vi "Camera Messenger.vi"(0 "Notifier Name":string, 1 "Binning":u16, 2 "General Camera Actions":T3, 5 "Exposure Time (s)":dbl, 7 "Save Path":path, 9 "No. of Frames":u32, 11 "Camera ROI":T1, 12 "Cooler On/Off":bool, 13 "Defect Correction On/Off":bool, 14 "Fan On/Off":bool) -> (3 "Current Exposure Time (s)":dbl, 4 "Notifier Name Dup":string, 6 "Running?":bool, 8 "Camera ROI":T1, 10 "Current Frame":u32, 15 "Image Ref":T2)   [LabVIEW 2021]
uses:
  Camera Controls/Generic Camera Actions.ctl
  Camera Controls/Generic Camera ROI.ctl
  <vilib>/vision/Image Controls.llb/IMAQ Image.ctl
  Hardware Configuration/Hardware Configuration Controls/Company.ctl
  Hamamatsu/Orca Flash/Orca Flash Controls/Orca Flash ROI.ctl
  Hamamatsu/Orca Flash/Orca Flash Controls/Orca Flash Parameters.ctl
  Hamamatsu/Orca Flash/Orca Flash Controls/Orca Flash Parameter List.ctl
  Hamamatsu/Orca Flash/Orca Flash Controls/Orca Flash Actions.ctl
  IDS/IDS Controls/IDS ROI.ctl
  IDS/IDS Controls/IDS Parameters.ctl
  IDS/IDS Controls/IDS Parameter List.ctl
  IDS/IDS Controls/IDS Actions.ctl
  Ximea/Ximea Controls/Ximea ROI.ctl
  Ximea/Ximea Controls/Ximea Parameters.ctl
  Ximea/Ximea Controls/Ximea Parameter List.ctl
  Ximea/Ximea Controls/Ximea Actions.ctl
  Photometrics/Prime BSI/R Cubed SITK/Prime BSI R3 Controls/Prime R3 ROI.ctl
  Photometrics/Prime BSI/R Cubed SITK/Prime BSI R3 Controls/Prime R3 Parameters.ctl
  Photometrics/Prime BSI/R Cubed SITK/Prime BSI R3 Controls/Prime R3 Parameter List.ctl
  Photometrics/Prime BSI/R Cubed SITK/Prime BSI R3 Controls/Prime R3 Actions.ctl
  Camera Controls/Camera IMAQ Key Info.ctl
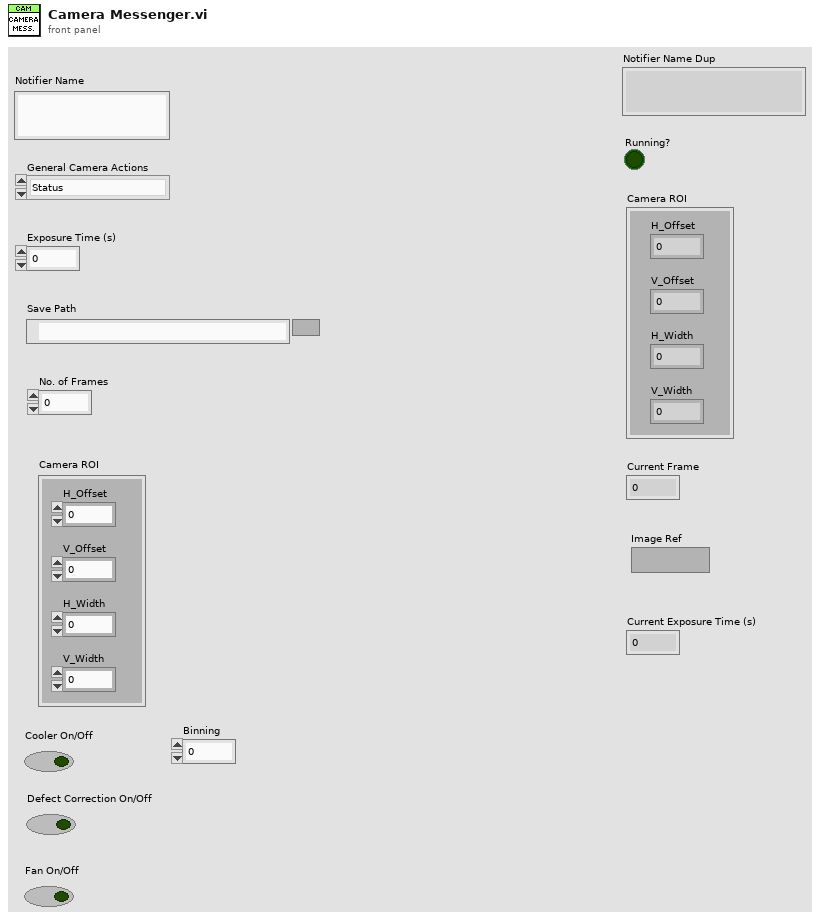
[diagram p1: front panel]
types:
  T1 = typedef "Generic Camera ROI.ctl" = cluster{"H_Offset":u16, "V_Offset":u16, "H_Width":u16, "V_Width":u16}
  T2 = typedef "IMAQ Image.ctl" = refnum<image>
  T3 = typedef "Generic Camera Actions.ctl" = enum16{"Status", "Live Preview", "Capture", "Abort", "Set Exposure Time (s)", "Get Exposure Time (s)", "Set Gain", "Get Gain", "Set Gamma", "Get Gamma", "Record Settings", "Set ROI", "Get ROI", "Binning", "Defect Correction On/Off", "Cooler On/Off", "Fan On/Off", "Quit"}
  T4 = typedef "Company.ctl" = enum16{"AA Opto Electronic", "ASI", "Coherent", "CVI", "DAQmx", "Hamamatsu", "IDS", "Ximea", "Mad City Labs", "Marzhauser", "Measurement Computing", "MPB Com", "Photometrics", "PI", "Prior", "Thorlabs"}
  T5 = typedef "Orca Flash Parameters.ctl" = cluster{"Value":dbl, "Orca Flash Parameters":T6}
  T6 = typedef "Orca Flash Parameter List.ctl" = u32
  T7 = typedef "Orca Flash ROI.ctl" = cluster{"H Offset":i32, "V Offset":i32, "H Width":i32, "V Width":i32}
  T8 = typedef "Orca Flash Actions.ctl" = enum16{"IDLE", "PREVIEW", "RECORD", "Send Trigger", "SOFT TRIGGER", "Record Settings", "SETPARAM", "GETPARAM", "SETROI", "GETROI", "PROGRESSIVE MODE", "AREA MODE", "STATUS", "QUIT"}
  T9 = typedef "IDS Parameter List.ctl" = enum16{"Exposure Time (s)", "Binning", "Gain", "Gamma"}
  T10 = typedef "IDS Parameters.ctl" = cluster{"Parameter":T9, "Value":dbl}
  T11 = typedef "IDS ROI.ctl" = cluster{"H Offset":i32, "V Offset":i32, "H Width":i32, "V Width":i32}
  T12 = typedef "IDS Actions.ctl" = enum16{"Error Check", "Initialize", "Preview", "Record", "Abort", "Record Settings", "Set Parameter", "Get Parameter", "Set ROI", "Get ROI", "Status", "Quit"}
  T13 = typedef "Ximea Parameter List.ctl" = enum16{"Exposure Time (s)", "Gain"}
  T14 = typedef "Ximea Parameters.ctl" = cluster{"Parameter":T13, "Value":sgl}
  T15 = typedef "Ximea ROI.ctl" = cluster{"H Offset":i32, "V Offset":i32, "H Width":i32, "V Width":i32}
  T16 = typedef "Ximea Actions.ctl" = enum16{"Idle", "Error Check", "Preview", "Record", "Soft Trigger", "Abort", "Record Settings", "Set Parameter", "Get Parameter", "Set ROI", "Get ROI", "Status", "Quit"}
  T17 = typedef "Prime R3 Parameter List.ctl" = enum16{"Exposure Time (s)"}
  T18 = typedef "Prime R3 Parameters.ctl" = cluster{"Parameter":T17, "Value":dbl}
  T19 = typedef "Prime R3 ROI.ctl" = cluster{"X Start":u32, "X End":u32, "X Bin":u32, "Y Start":u32, "Y End":u32, "Y Bin":u32}
  T20 = typedef "Prime R3 Actions.ctl" = enum16{"Error Check", "Initialize", "Preview", "Record", "Abort", "Record Settings", "Set Parameter", "Get Parameter", "Set ROI", "Get ROI", "Status", "Set Trigger", "Quit"}
  T21 = typedef "Camera IMAQ Key Info.ctl" = cluster{"Frame":u32, "Sensor Height":i32, "Sensor Width":i32, "ROI Height":i32, "ROI Width":i32, "ROI Enable?":bool, "Bit per Pixel":u8}
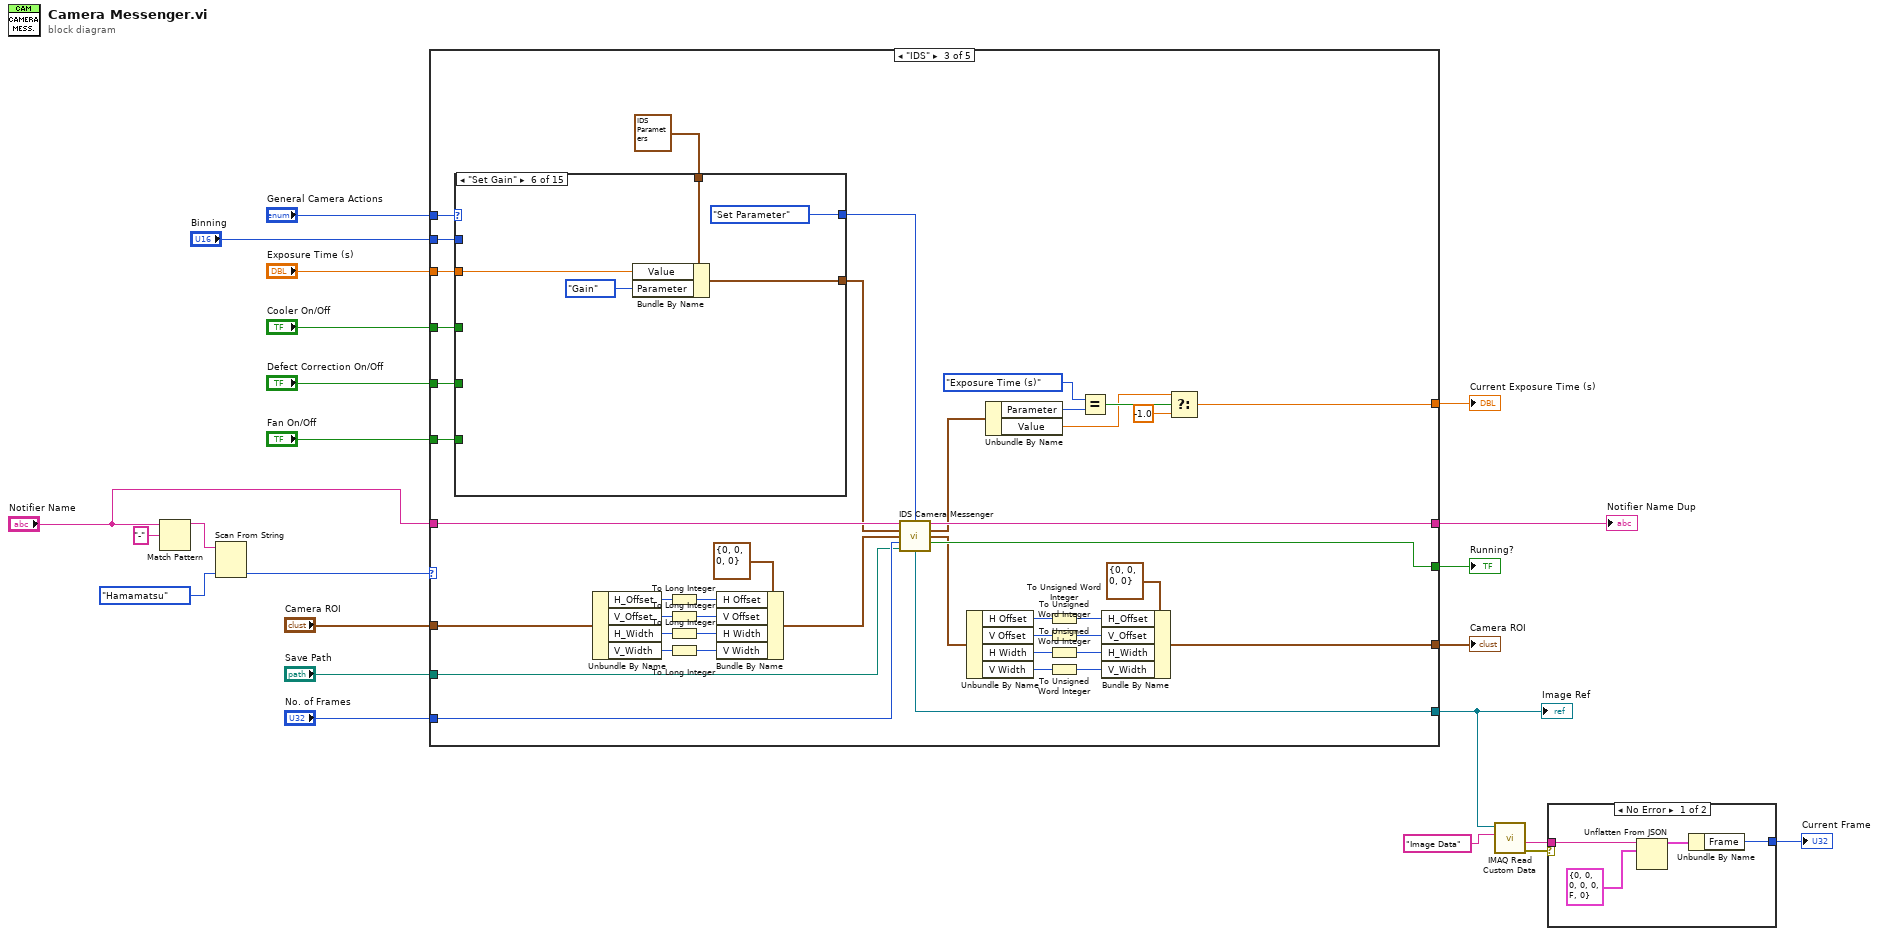
[diagram p0: block diagram]
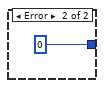
[diagram p2: hidden frame]
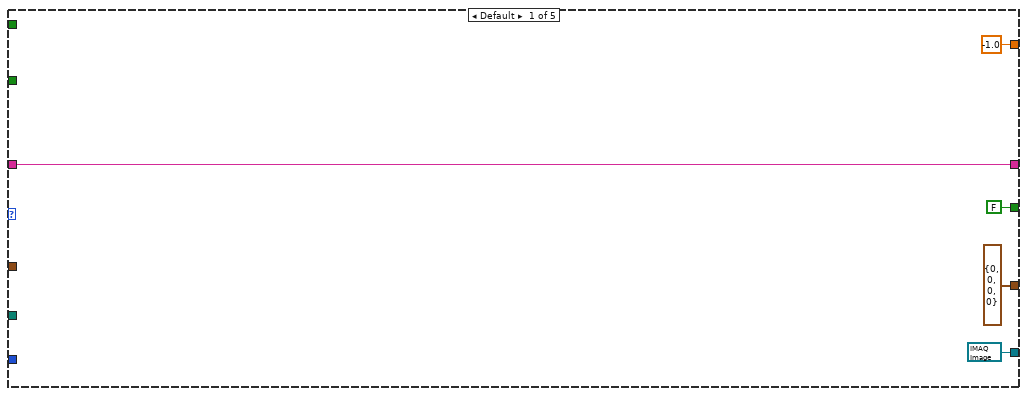
[diagram p3: hidden frame]
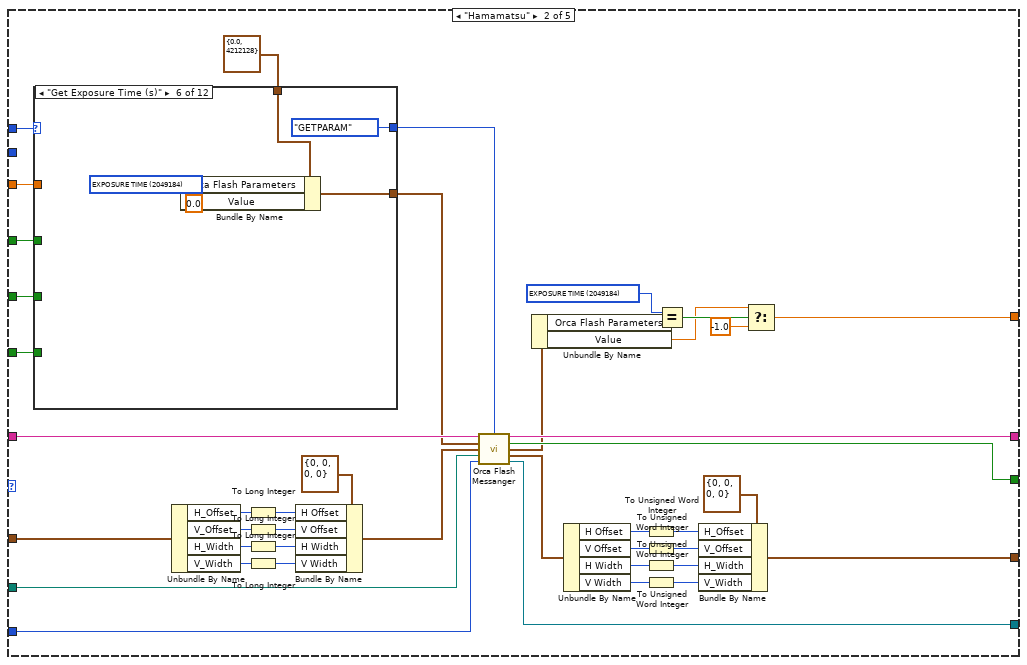
[diagram p4: hidden frame]
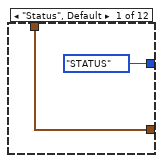
[diagram p5: hidden frame]
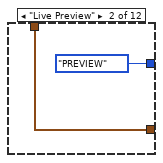
[diagram p6: hidden frame]
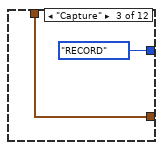
[diagram p7: hidden frame]
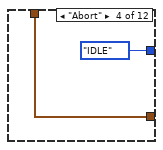
[diagram p8: hidden frame]
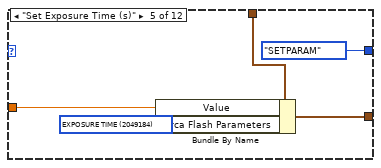
[diagram p9: hidden frame]
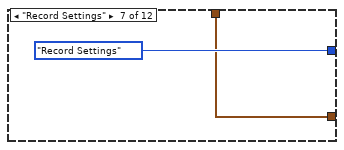
[diagram p10: hidden frame]
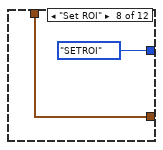
[diagram p11: hidden frame]
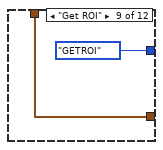
[diagram p12: hidden frame]
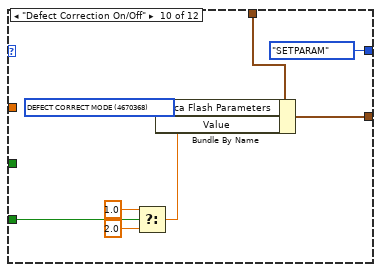
[diagram p13: hidden frame]
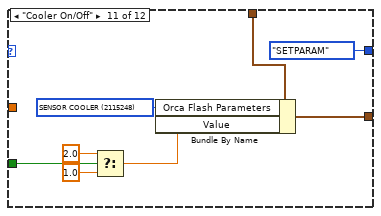
[diagram p14: hidden frame]
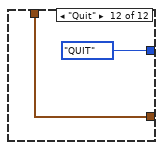
[diagram p15: hidden frame]
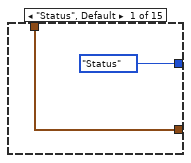
[diagram p16: hidden frame]
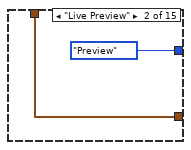
[diagram p17: hidden frame]
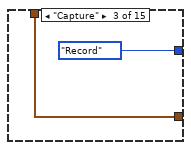
[diagram p18: hidden frame]
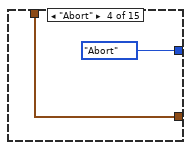
[diagram p19: hidden frame]
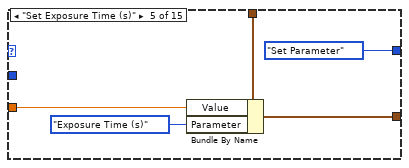
[diagram p20: hidden frame]
diagram:
  n1 = Match Pattern(string="Notifier Name", regular expression="-") -> (before substring=w20:string)  [unwired: 1 in, 3 out]
  n2 = Scan From String(input string=w20, default 1=Company."Hamamatsu" ("Company")) -> (output 1=w21:T4)  [unwired: 3 in, 3 out]
  n3 = case shown="\"IDS\"" w21 {
    tunnel: "Notifier Name" -> [w28 w71 w157 w246 w318]
    tunnel: "General Camera Actions" -> [_ w56 w142 w231 w311]
    tunnel: "No. of Frames" -> [_ w70 w156 w245 w317]
    tunnel: "Save Path" -> [_ w69 w155 w244 w289]
    tunnel: "Camera ROI" -> [_ w67 w153 w242 w315]
    tunnel: [w28 w57 w143 w232 w312] -> w15
    tunnel: "Exposure Time (s)" -> [_ w51 w138 w227 w307]
    tunnel: "Cooler On/Off" -> [_ w55 w141 w230 w310]
    tunnel: "Defect Correction On/Off" -> [_ w54 w140 w229 w309]
    tunnel: "Fan On/Off" -> [_ w53 w139 w228 w308]
    tunnel: [T2 refnum ("Image Ref") w48 w135 w224 w304] -> w6
    tunnel: [FALSE ("Running?") w47 w134 w223 w303] -> w10
    tunnel: [T1 {"H_Offset"=0, "V_Offset"=0, "H_Width"=0, "V_Width"=0} ("General Camera ROI") w36 w123 w212 w292] -> w9
    tunnel: [-1.0 ("f") w30 w115 w206 w274] -> w2
    tunnel: "Binning" -> [_ _ w114 _ _]
    frame Default {
    }
    frame "Hamamatsu" {
      w29 = T6 2049184 items=["SENSOR MODE"=4212128, "READOUT SPEED"=4211872, "READOUT DIRECTION"=4211904, "TRIGGER GLOBAL EXPOSURE"=2049680, "TRIGGER DELAY"=1066480, "SYNC READOUT SYSTEM BLANK"=1066528, "SENSOR COOLER"=2115248, "SENSOR COOLER STATUS"=2115280, "EXPOSURE TIME"=2049184, "DEFECT CORRECT MODE"=4670368, "BINNING"=4215968, "INTERNAL LINE SPEED"=4226000, "INTERNAL LINE INTERVAL"=4226016, "IMAGE PIXEL TYPE"=4343296, "NUMBER OF OUTPUT TRIGGER CONNECTOR"=1852320, "OUTPUT TRIGGER SOURCE[0]"=1852576, "OUTPUT TRIGGER SOURCE[1]"=1852832, "OUTPUT TRIGGER SOURCE[2]"=1853088, "OUTPUT TRIGGER POLARITY[0]"=1852592, "OUTPUT TRIGGER POLARITY[1]"=1852848, "OUTPUT TRIGGER POLARITY[2]"=1853104, "OUTPUT TRIGGER ACTIVE[0]"=1852608, "OUTPUT TRIGGER ACTIVE[1]"=1852864, "OUTPUT TRIGGER ACTIVE[2]"=1853120, "OUTPUT TRIGGER DELAY[0]"=1852624, "OUTPUT TRIGGER DELAY[1]"=1852880, "OUTPUT TRIGGER DELAY[2]"=1853136, "OUTPUT TRIGGER PERIOD[0]"=1852640, "OUTPUT TRIGGER PERIOD[1]"=1852896, "OUTPUT TRIGGER PERIOD[2]"=1853152, "OUTPUT TRIGGER KIND[0]"=1852656, "OUTPUT TRIGGER KIND[1]"=1852912, "OUTPUT TRIGGER KIND[2]"=1853168, "OUTPUT TRIGGER PRE HSYNC COUNT"=1852704] ("x")
      n4 = case shown="\"Get Exposure Time (s)\"" w56 {
        tunnel: w55 -> [_ _ _ _ _ _ _ _ _ _ w108 _]
        tunnel: w54 -> [_ _ _ _ _ _ _ _ _ w99 _ _]
        tunnel: w53 -> [_ _ _ _ _ _ _ _ _ _ _ _]
        tunnel: [Orca_Flash_Actions."STATUS" ("Camera Actions") Orca_Flash_Actions."PREVIEW" ("Camera Actions") Orca_Flash_Actions."RECORD" ("Camera Actions") Orca_Flash_Actions."IDLE" ("Camera Actions") Orca_Flash_Actions."SETPARAM" ("Camera Actions") Orca_Flash_Actions."GETPARAM" ("Camera Actions") Orca_Flash_Actions."Record Settings" ("Camera Actions") Orca_Flash_Actions."SETROI" ("Camera Actions") Orca_Flash_Actions."GETROI" ("Camera Actions") Orca_Flash_Actions."SETPARAM" ("Camera Actions") Orca_Flash_Actions."SETPARAM" ("Camera Actions") Orca_Flash_Actions."QUIT" ("Camera Actions")] -> w52
        tunnel: w51 -> [_ _ _ _ w83 _ _ _ _ _ _ _]
        tunnel: [w72 w74 w76 w78 w82 w88 w90 w92 w94 w101 w104 w113] -> w50
        tunnel: T5 {"Value"=0.0, "Orca Flash Parameters"=4212128} ("sCMOS Parameter") -> [w72 w74 w76 w78 w81 w89 w90 w92 w94 w102 w110 w113]
        frame "Status", Default {
        }
        frame "Live Preview" {
        }
        frame "Capture" {
        }
        frame "Abort" {
        }
        frame "Set Exposure Time (s)" {
          w80 = T6 2049184 items=["SENSOR MODE"=4212128, "READOUT SPEED"=4211872, "READOUT DIRECTION"=4211904, "TRIGGER GLOBAL EXPOSURE"=2049680, "TRIGGER DELAY"=1066480, "SYNC READOUT SYSTEM BLANK"=1066528, "SENSOR COOLER"=2115248, "SENSOR COOLER STATUS"=2115280, "EXPOSURE TIME"=2049184, "DEFECT CORRECT MODE"=4670368, "BINNING"=4215968, "INTERNAL LINE SPEED"=4226000, "INTERNAL LINE INTERVAL"=4226016, "IMAGE PIXEL TYPE"=4343296, "NUMBER OF OUTPUT TRIGGER CONNECTOR"=1852320, "OUTPUT TRIGGER SOURCE[0]"=1852576, "OUTPUT TRIGGER SOURCE[1]"=1852832, "OUTPUT TRIGGER SOURCE[2]"=1853088, "OUTPUT TRIGGER POLARITY[0]"=1852592, "OUTPUT TRIGGER POLARITY[1]"=1852848, "OUTPUT TRIGGER POLARITY[2]"=1853104, "OUTPUT TRIGGER ACTIVE[0]"=1852608, "OUTPUT TRIGGER ACTIVE[1]"=1852864, "OUTPUT TRIGGER ACTIVE[2]"=1853120, "OUTPUT TRIGGER DELAY[0]"=1852624, "OUTPUT TRIGGER DELAY[1]"=1852880, "OUTPUT TRIGGER DELAY[2]"=1853136, "OUTPUT TRIGGER PERIOD[0]"=1852640, "OUTPUT TRIGGER PERIOD[1]"=1852896, "OUTPUT TRIGGER PERIOD[2]"=1853152, "OUTPUT TRIGGER KIND[0]"=1852656, "OUTPUT TRIGGER KIND[1]"=1852912, "OUTPUT TRIGGER KIND[2]"=1853168, "OUTPUT TRIGGER PRE HSYNC COUNT"=1852704] ("Parameter")
          n5 = Bundle By Name(cluster=w81, "Value"=w83, "Orca Flash Parameters"=w80) -> (w82:T5)
        }
        frame "Get Exposure Time (s)" {
          w86 = T6 2049184 items=["SENSOR MODE"=4212128, "READOUT SPEED"=4211872, "READOUT DIRECTION"=4211904, "TRIGGER GLOBAL EXPOSURE"=2049680, "TRIGGER DELAY"=1066480, "SYNC READOUT SYSTEM BLANK"=1066528, "SENSOR COOLER"=2115248, "SENSOR COOLER STATUS"=2115280, "EXPOSURE TIME"=2049184, "DEFECT CORRECT MODE"=4670368, "BINNING"=4215968, "INTERNAL LINE SPEED"=4226000, "INTERNAL LINE INTERVAL"=4226016, "IMAGE PIXEL TYPE"=4343296, "NUMBER OF OUTPUT TRIGGER CONNECTOR"=1852320, "OUTPUT TRIGGER SOURCE[0]"=1852576, "OUTPUT TRIGGER SOURCE[1]"=1852832, "OUTPUT TRIGGER SOURCE[2]"=1853088, "OUTPUT TRIGGER POLARITY[0]"=1852592, "OUTPUT TRIGGER POLARITY[1]"=1852848, "OUTPUT TRIGGER POLARITY[2]"=1853104, "OUTPUT TRIGGER ACTIVE[0]"=1852608, "OUTPUT TRIGGER ACTIVE[1]"=1852864, "OUTPUT TRIGGER ACTIVE[2]"=1853120, "OUTPUT TRIGGER DELAY[0]"=1852624, "OUTPUT TRIGGER DELAY[1]"=1852880, "OUTPUT TRIGGER DELAY[2]"=1853136, "OUTPUT TRIGGER PERIOD[0]"=1852640, "OUTPUT TRIGGER PERIOD[1]"=1852896, "OUTPUT TRIGGER PERIOD[2]"=1853152, "OUTPUT TRIGGER KIND[0]"=1852656, "OUTPUT TRIGGER KIND[1]"=1852912, "OUTPUT TRIGGER KIND[2]"=1853168, "OUTPUT TRIGGER PRE HSYNC COUNT"=1852704] ("Parameter")
          n6 = Bundle By Name(cluster=w89, "Orca Flash Parameters"=w86, "Value"=0.0) -> (w88:T5)
        }
        frame "Record Settings" {
        }
        frame "Set ROI" {
        }
        frame "Get ROI" {
        }
        frame "Defect Correction On/Off" {
          w100 = T6 4670368 items=["SENSOR MODE"=4212128, "READOUT SPEED"=4211872, "READOUT DIRECTION"=4211904, "TRIGGER GLOBAL EXPOSURE"=2049680, "TRIGGER DELAY"=1066480, "SYNC READOUT SYSTEM BLANK"=1066528, "SENSOR COOLER"=2115248, "SENSOR COOLER STATUS"=2115280, "EXPOSURE TIME"=2049184, "DEFECT CORRECT MODE"=4670368, "BINNING"=4215968, "INTERNAL LINE SPEED"=4226000, "INTERNAL LINE INTERVAL"=4226016, "IMAGE PIXEL TYPE"=4343296, "NUMBER OF OUTPUT TRIGGER CONNECTOR"=1852320, "OUTPUT TRIGGER SOURCE[0]"=1852576, "OUTPUT TRIGGER SOURCE[1]"=1852832, "OUTPUT TRIGGER SOURCE[2]"=1853088, "OUTPUT TRIGGER POLARITY[0]"=1852592, "OUTPUT TRIGGER POLARITY[1]"=1852848, "OUTPUT TRIGGER POLARITY[2]"=1853104, "OUTPUT TRIGGER ACTIVE[0]"=1852608, "OUTPUT TRIGGER ACTIVE[1]"=1852864, "OUTPUT TRIGGER ACTIVE[2]"=1853120, "OUTPUT TRIGGER DELAY[0]"=1852624, "OUTPUT TRIGGER DELAY[1]"=1852880, "OUTPUT TRIGGER DELAY[2]"=1853136, "OUTPUT TRIGGER PERIOD[0]"=1852640, "OUTPUT TRIGGER PERIOD[1]"=1852896, "OUTPUT TRIGGER PERIOD[2]"=1853152, "OUTPUT TRIGGER KIND[0]"=1852656, "OUTPUT TRIGGER KIND[1]"=1852912, "OUTPUT TRIGGER KIND[2]"=1853168, "OUTPUT TRIGGER PRE HSYNC COUNT"=1852704] ("Parameter")
          n7 = Select(t=1.0, s=w99, f=2.0) -> (s? t:f=w96:dbl)
          n8 = Bundle By Name(cluster=w102, "Orca Flash Parameters"=w100, "Value"=w96) -> (w101:T5)
        }
        frame "Cooler On/Off" {
          w109 = T6 2115248 items=["SENSOR MODE"=4212128, "READOUT SPEED"=4211872, "READOUT DIRECTION"=4211904, "TRIGGER GLOBAL EXPOSURE"=2049680, "TRIGGER DELAY"=1066480, "SYNC READOUT SYSTEM BLANK"=1066528, "SENSOR COOLER"=2115248, "SENSOR COOLER STATUS"=2115280, "EXPOSURE TIME"=2049184, "DEFECT CORRECT MODE"=4670368, "BINNING"=4215968, "INTERNAL LINE SPEED"=4226000, "INTERNAL LINE INTERVAL"=4226016, "IMAGE PIXEL TYPE"=4343296, "NUMBER OF OUTPUT TRIGGER CONNECTOR"=1852320, "OUTPUT TRIGGER SOURCE[0]"=1852576, "OUTPUT TRIGGER SOURCE[1]"=1852832, "OUTPUT TRIGGER SOURCE[2]"=1853088, "OUTPUT TRIGGER POLARITY[0]"=1852592, "OUTPUT TRIGGER POLARITY[1]"=1852848, "OUTPUT TRIGGER POLARITY[2]"=1853104, "OUTPUT TRIGGER ACTIVE[0]"=1852608, "OUTPUT TRIGGER ACTIVE[1]"=1852864, "OUTPUT TRIGGER ACTIVE[2]"=1853120, "OUTPUT TRIGGER DELAY[0]"=1852624, "OUTPUT TRIGGER DELAY[1]"=1852880, "OUTPUT TRIGGER DELAY[2]"=1853136, "OUTPUT TRIGGER PERIOD[0]"=1852640, "OUTPUT TRIGGER PERIOD[1]"=1852896, "OUTPUT TRIGGER PERIOD[2]"=1853152, "OUTPUT TRIGGER KIND[0]"=1852656, "OUTPUT TRIGGER KIND[1]"=1852912, "OUTPUT TRIGGER KIND[2]"=1853168, "OUTPUT TRIGGER PRE HSYNC COUNT"=1852704] ("Parameter")
          n9 = Select(t=2.0, s=w108, f=1.0) -> (s? t:f=w105:dbl)
          n10 = Bundle By Name(cluster=w110, "Orca Flash Parameters"=w109, "Value"=w105) -> (w104:T5)
        }
        frame "Quit" {
        }
      }
      n11 = Unbundle By Name(w67) -> ("H_Offset"=w63:u16, "V_Offset"=w64:u16, "H_Width"=w65:u16, "V_Width"=w66:u16)
      n12 = To Long Integer(number=w63) -> (32bit integer=w62:i32)
      n13 = To Long Integer(number=w64) -> (32bit integer=w61:i32)
      n14 = To Long Integer(number=w65) -> (32bit integer=w60:i32)
      n15 = To Long Integer(number=w66) -> (32bit integer=w59:i32)
      n16 = Bundle By Name(cluster=T7 {"H Offset"=0, "V Offset"=0, "H Width"=0, "V Width"=0} ("sCMOS ROI"), "H Offset"=w62, "V Offset"=w61, "H Width"=w60, "V Width"=w59) -> (w58:T7)
      n17 = call "Orca Flash Messanger.vi"("Notifier Name"=w71, "Camera Actions"=w52, "sCMOS Parameter"=w50, "sCMOS ROI"=w58, "Path"=w69, "# of frames"=w70) -> ("Notifier Name Dup"=w57:string, "Running?"=w47:bool, "sCMOS Parameter"=w31:T5, "sCMOS ROI"=w45:T7, "Image Ref"=w48:T2)  [unwired: 5 in]
      n18 = Unbundle By Name(w31) -> ("Orca Flash Parameters"=w35:T6, "Value"=w33:dbl)
      n19 = Unbundle By Name(w45) -> ("H Offset"=w44:i32, "V Offset"=w43:i32, "H Width"=w42:i32, "V Width"=w41:i32)
      n20 = To Unsigned Word Integer(number=w44) -> (unsigned 16bit integer=w40:u16)
      n21 = To Unsigned Word Integer(number=w43) -> (unsigned 16bit integer=w39:u16)
      n22 = To Unsigned Word Integer(number=w42) -> (unsigned 16bit integer=w38:u16)
      n23 = To Unsigned Word Integer(number=w41) -> (unsigned 16bit integer=w37:u16)
      n24 = Equal?(x=w29, y=w35) -> (x = y?=w34:bool)
      n25 = Bundle By Name(cluster=T1 {"H_Offset"=0, "V_Offset"=0, "H_Width"=0, "V_Width"=0} ("General Camera ROI"), "H_Offset"=w40, "V_Offset"=w39, "H_Width"=w38, "V_Width"=w37) -> (w36:T1)
      n26 = Select(t=w33, s=w34, f=-1.0) -> (s? t:f=w30:dbl)
    }
    frame "IDS" {
      n27 = case shown="\"Set Gain\"" w142 {
        tunnel: w141 -> [_ _ _ _ _ _ _ _ _ _ _ _ _ _ _]
        tunnel: w140 -> [_ _ _ _ _ _ _ _ _ _ _ _ _ _ _]
        tunnel: w139 -> [_ _ _ _ _ _ _ _ _ _ _ _ _ _ _]
        tunnel: [IDS_Actions."Status" ("IDS Actions") IDS_Actions."Preview" ("IDS Actions") IDS_Actions."Record" ("IDS Actions") IDS_Actions."Abort" ("IDS Actions") IDS_Actions."Set Parameter" ("IDS Actions") IDS_Actions."Set Parameter" ("IDS Actions") IDS_Actions."Set Parameter" ("IDS Actions") IDS_Actions."Get Parameter" ("IDS Actions") IDS_Actions."Record Settings" ("IDS Actions") IDS_Actions."Set ROI" ("IDS Actions") IDS_Actions."Get ROI" ("IDS Actions") IDS_Actions."Set Parameter" ("IDS Actions") IDS_Actions."Status" ("IDS Actions") IDS_Actions."Status" ("IDS Actions") IDS_Actions."Quit" ("IDS Actions")] -> w122
        tunnel: w138 -> [_ _ _ _ w170 w171 w176 _ _ _ _ _ _ _ _]
        tunnel: [w159 w161 w163 w165 w169 w175 w180 w181 w187 w189 w191 w193 w199 w201 w203] -> w137
        tunnel: T10 {"Parameter"=enum."Exposure Time (s)", "Value"=4212128.0} ("IDS Parameter") -> [w159 w161 w163 w165 w168 w174 w179 w184 w187 w189 w191 w192 w199 w201 w203]
        tunnel: w114 -> [_ _ _ _ _ _ _ _ _ _ _ w195 _ _ _]
        frame "Status", Default {
        }
        frame "Live Preview" {
        }
        frame "Capture" {
        }
        frame "Abort" {
        }
        frame "Set Exposure Time (s)" {
          n28 = Bundle By Name(cluster=w168, "Value"=w170, "Parameter"=IDS_Parameter_List."Exposure Time (s)") -> (w169:T10)
        }
        frame "Set Gain" {
          n29 = Bundle By Name(cluster=w174, "Value"=w171, "Parameter"=IDS_Parameter_List."Gain") -> (w175:T10)
        }
        frame "Set Gamma" {
          n30 = Bundle By Name(cluster=w179, "Value"=w176, "Parameter"=IDS_Parameter_List."Gamma") -> (w180:T10)
        }
        frame "Get Exposure Time (s)" {
          n31 = Bundle By Name(cluster=w184, "Parameter"=IDS_Parameter_List."Exposure Time (s)", "Value"=0.0) -> (w181:T10)
        }
        frame "Record Settings" {
        }
        frame "Set ROI" {
        }
        frame "Get ROI" {
        }
        frame "Binning" {
          n32 = To Double Precision Float(number=w195) -> (double precision float=w196:dbl)
          n33 = Bundle By Name(cluster=w192, "Parameter"=IDS_Parameter_List."Binning", "Value"=w196) -> (w193:T10)
        }
        frame "Defect Correction On/Off" {
        }
        frame "Cooler On/Off" {
        }
        frame "Quit" {
        }
      }
      n34 = Unbundle By Name(w153) -> ("H_Offset"=w149:u16, "V_Offset"=w150:u16, "H_Width"=w151:u16, "V_Width"=w152:u16)
      n35 = To Long Integer(number=w149) -> (32bit integer=w148:i32)
      n36 = To Long Integer(number=w150) -> (32bit integer=w147:i32)
      n37 = To Long Integer(number=w151) -> (32bit integer=w146:i32)
      n38 = To Long Integer(number=w152) -> (32bit integer=w145:i32)
      n39 = Bundle By Name(cluster=T11 {"H Offset"=0, "V Offset"=0, "H Width"=0, "V Width"=0} ("sCMOS ROI"), "H Offset"=w148, "V Offset"=w147, "H Width"=w146, "V Width"=w145) -> (w144:T11)
      n40 = call "IDS Camera Messenger.vi"("Notifier Name"=w157, "IDS Actions"=w122, "IDS Parameter"=w137, "ROI Setup"=w144, "# of Frames"=w156, "File Save Path"=w155) -> ("Notifier Name (Dup)"=w143:string, "IDS Parameter"=w121:T10, "IDS ROI"=w132:T11, "Running?"=w134:bool, "Image Ref"=w135:T2)  [unwired: 4 in, 1 out]
      n41 = Unbundle By Name(w132) -> ("H Offset"=w131:i32, "V Offset"=w130:i32, "H Width"=w129:i32, "V Width"=w128:i32)
      n42 = Unbundle By Name(w121) -> ("Parameter"=w120:T9, "Value"=w117:dbl)
      n43 = To Unsigned Word Integer(number=w131) -> (unsigned 16bit integer=w127:u16)
      n44 = To Unsigned Word Integer(number=w130) -> (unsigned 16bit integer=w126:u16)
      n45 = To Unsigned Word Integer(number=w129) -> (unsigned 16bit integer=w125:u16)
      n46 = To Unsigned Word Integer(number=w128) -> (unsigned 16bit integer=w124:u16)
      n47 = Equal?(x=IDS_Parameter_List."Exposure Time (s)", y=w120) -> (x = y?=w118:bool)
      n48 = Bundle By Name(cluster=T1 {"H_Offset"=0, "V_Offset"=0, "H_Width"=0, "V_Width"=0} ("General Camera ROI"), "H_Offset"=w127, "V_Offset"=w126, "H_Width"=w125, "V_Width"=w124) -> (w123:T1)
      n49 = Select(t=w117, s=w118, f=-1.0) -> (s? t:f=w115:dbl)
    }
    frame "Ximea" {
      n50 = case shown="\"Abort\"" w231 {
        tunnel: w230 -> [_ _ _ _ _ _ _ _ _ _]
        tunnel: w229 -> [_ _ _ _ _ _ _ _ _ _]
        tunnel: w228 -> [_ _ _ _ _ _ _ _ _ _]
        tunnel: w227 -> [_ _ _ _ w256 _ _ _ _ _]
        tunnel: [w248 w250 w252 w254 w260 w263 w266 w268 w270 w272] -> w226
        tunnel: T14 {"Parameter"=enum."Exposure Time (s)", "Value"=4212128.0} ("Ximea  Parameter") -> [w248 w250 w252 w254 w259 w264 w266 w268 w270 w272]
        tunnel: [Ximea_Actions."Status" ("Ximea Actions") Ximea_Actions."Preview" ("Ximea Actions") Ximea_Actions."Record" ("Ximea Actions") Ximea_Actions."Idle" ("Ximea Actions") Ximea_Actions."Set Parameter" ("Ximea Actions") Ximea_Actions."Get Parameter" ("Ximea Actions") Ximea_Actions."Record Settings" ("Ximea Actions") Ximea_Actions."Set ROI" ("Ximea Actions") Ximea_Actions."Get ROI" ("Ximea Actions") Ximea_Actions."Quit" ("Ximea Actions")] -> w205
        frame "Status", Default {
        }
        frame "Live Preview" {
        }
        frame "Capture" {
        }
        frame "Abort" {
        }
        frame "Set Exposure Time (s)" {
          n51 = To Single Precision Float(number=w256) -> (single precision float=w255:sgl)
          n52 = Bundle By Name(cluster=w259, "Value"=w255, "Parameter"=Ximea_Parameter_List."Exposure Time (s)") -> (w260:T14)
        }
        frame "Get Exposure Time (s)" {
          n53 = Bundle By Name(cluster=w264, "Parameter"=Ximea_Parameter_List."Exposure Time (s)") -> (w263:T14)
        }
        frame "Record Settings" {
        }
        frame "Set ROI" {
        }
        frame "Get ROI" {
        }
        frame "Quit" {
        }
      }
      n54 = Unbundle By Name(w242) -> ("H_Offset"=w238:u16, "V_Offset"=w239:u16, "H_Width"=w240:u16, "V_Width"=w241:u16)
      n55 = To Long Integer(number=w238) -> (32bit integer=w237:i32)
      n56 = To Long Integer(number=w239) -> (32bit integer=w236:i32)
      n57 = To Long Integer(number=w240) -> (32bit integer=w235:i32)
      n58 = To Long Integer(number=w241) -> (32bit integer=w234:i32)
      n59 = Bundle By Name(cluster=T15 {"H Offset"=0, "V Offset"=0, "H Width"=0, "V Width"=0} ("sCMOS ROI"), "H Offset"=w237, "V Offset"=w236, "H Width"=w235, "V Width"=w234) -> (w233:T15)
      n60 = call "Ximea Camera Messenger.vi"("Notifier Name"=w246, "Ximea Actions"=w205, "Ximea  Parameter"=w226, "ROI Setup"=w233, "# of Frames"=w245, "File Save Path"=w244) -> ("Notifier Name (Dup)"=w232:string, "Running?"=w223:bool, "Ximea Parameter Out"=w211:T14, "Ximea ROI Out"=w221:T15, "Image Ref"=w224:T2)  [unwired: 5 in]
      n61 = Unbundle By Name(w211) -> ("Parameter"=w210:T13, "Value"=w208:sgl)
      n62 = Unbundle By Name(w221) -> ("H Offset"=w220:i32, "V Offset"=w219:i32, "H Width"=w218:i32, "V Width"=w217:i32)
      n63 = To Unsigned Word Integer(number=w220) -> (unsigned 16bit integer=w216:u16)
      n64 = To Unsigned Word Integer(number=w219) -> (unsigned 16bit integer=w215:u16)
      n65 = To Unsigned Word Integer(number=w218) -> (unsigned 16bit integer=w214:u16)
      n66 = To Unsigned Word Integer(number=w217) -> (unsigned 16bit integer=w213:u16)
      n67 = Equal?(x=Ximea_Parameter_List."Exposure Time (s)", y=w210) -> (x = y?=w209:bool)
      n68 = Bundle By Name(cluster=T1 {"H_Offset"=0, "V_Offset"=0, "H_Width"=0, "V_Width"=0} ("General Camera ROI"), "H_Offset"=w216, "V_Offset"=w215, "H_Width"=w214, "V_Width"=w213) -> (w212:T1)
      n69 = Select(t=w208, s=w209, f=-1.0) -> (s? t:f=w206:dbl)
    }
    frame "Photometrics" {
      w290 = u32 1 ("number")
      n70 = case shown="\"Status\", Default" w311 {
        tunnel: w310 -> [_ _ _ _ _ _ _ _ _ _ _ _]
        tunnel: w309 -> [_ _ _ _ _ _ _ _ _ _ _ _]
        tunnel: w308 -> [_ _ _ _ _ _ _ _ _ _ _ _]
        tunnel: [Prime_R3_Actions."Status" ("Prime Actions") Prime_R3_Actions."Preview" ("Prime Actions") Prime_R3_Actions."Record" ("Prime Actions") Prime_R3_Actions."Abort" ("Prime Actions") Prime_R3_Actions."Set Parameter" ("Prime Actions") Prime_R3_Actions."Get Parameter" ("Prime Actions") Prime_R3_Actions."Record Settings" ("Prime Actions") Prime_R3_Actions."Set ROI" ("Prime Actions") Prime_R3_Actions."Get ROI" ("Prime Actions") Prime_R3_Actions."Status" ("Prime Actions") Prime_R3_Actions."Status" ("Prime Actions") Prime_R3_Actions."Quit" ("Prime Actions")] -> w291
        tunnel: w307 -> [_ _ _ _ w331 _ _ _ _ _ _ _]
        tunnel: [w320 w322 w324 w326 w330 w334 w338 w340 w342 w344 w346 w348] -> w306
        tunnel: T18 {"Parameter"=enum."Exposure Time (s)", "Value"=4212128.0} ("Prime Parameter") -> [w320 w322 w324 w326 w329 w335 w338 w340 w342 w344 w346 w348]
        frame "Status", Default {
        }
        frame "Live Preview" {
        }
        frame "Capture" {
        }
        frame "Abort" {
        }
        frame "Set Exposure Time (s)" {
          n71 = Bundle By Name(cluster=w329, "Value"=w331, "Parameter"=Prime_R3_Parameter_List."Exposure Time (s)") -> (w330:T18)
        }
        frame "Get Exposure Time (s)" {
          n72 = Bundle By Name(cluster=w335, "Parameter"=Prime_R3_Parameter_List."Exposure Time (s)", "Value"=0.0) -> (w334:T18)
        }
        frame "Record Settings" {
        }
        frame "Set ROI" {
        }
        frame "Get ROI" {
        }
        frame "Defect Correction On/Off" {
        }
        frame "Cooler On/Off" {
        }
        frame "Quit" {
        }
      }
      n73 = Unbundle By Name(w315) -> ("V_Offset"=w281:u16, "V_Width"=w283:u16, "H_Offset"=w287:u16, "H_Width"=w288:u16)
      n74 = Add(x=w281, y=w283) -> (x+y=w282:u16)
      n75 = Add(x=w287, y=w288) -> (x+y=w285:u16)
      n76 = To Unsigned Long Integer(number=w281) -> (unsigned 32bit integer=w280:u32)
      n77 = To Unsigned Long Integer(number=w282) -> (unsigned 32bit integer=w314:u32)
      n78 = To Unsigned Long Integer(number=w287) -> (unsigned 32bit integer=w286:u32)
      n79 = To Unsigned Long Integer(number=w285) -> (unsigned 32bit integer=w284:u32)
      n80 = Bundle By Name(cluster=T19 {"X Start"=0, "X End"=0, "X Bin"=0, "Y Start"=0, "Y End"=0, "Y Bin"=0} ("sCMOS ROI"), "X Start"=w280, "X End"=w314, "X Bin"=w290, "Y Start"=w286, "Y End"=w284, "Y Bin"=w290) -> (w313:T19)
      n81 = call "Prime BSI R3 Camera Messenger.vi"("Notifier Name"=w318, "Prime Actions"=w291, "Prime Parameter"=w306, "ROI Setup"=w313, "# of Frames"=w317, "File Save Path"=w289) -> ("Notifier Name (Dup)"=w312:string, "Prime Parameter"=w275:T18, "Prime ROI"=w301:T19, "Running?"=w303:bool, "Image Ref"=w304:T2)  [unwired: 4 in, 1 out]
      n82 = Unbundle By Name(w301) -> ("X Start"=w300:u32, "X End"=w299:u32, "X Bin"=w298:u32, "Y Start"=w297:u32)
      n83 = Unbundle By Name(w275) -> ("Parameter"=w279:T17, "Value"=w277:dbl)
      n84 = To Unsigned Word Integer(number=w300) -> (unsigned 16bit integer=w296:u16)
      n85 = To Unsigned Word Integer(number=w299) -> (unsigned 16bit integer=w295:u16)
      n86 = To Unsigned Word Integer(number=w298) -> (unsigned 16bit integer=w294:u16)
      n87 = To Unsigned Word Integer(number=w297) -> (unsigned 16bit integer=w293:u16)
      n88 = Bundle By Name(cluster=T1 {"H_Offset"=0, "V_Offset"=0, "H_Width"=0, "V_Width"=0} ("General Camera ROI"), "H_Offset"=w296, "V_Offset"=w295, "H_Width"=w294, "V_Width"=w293) -> (w292:T1)
      n89 = Equal?(x=Prime_R3_Parameter_List."Exposure Time (s)", y=w279) -> (x = y?=w278:bool)
      n90 = Select(t=w277, s=w278, f=-1.0) -> (s? t:f=w274:dbl)
    }
  }
  "Notifier Name Dup" <- w15
  "Image Ref" <- w6
  "Running?" <- w10
  "Camera ROI" <- w9
  "Current Exposure Time (s)" <- w2
  n91 = call "IMAQ Read Custom Data"("Key"="Image Data", "Image"=w6) -> ("error out"=w5:errorcluster, "Custom Data Out"=w7:string)  [unwired: 7 in, 1 out]
  n92 = case shown="No Error" w5 {
    tunnel: w7 -> [w352 _]
    tunnel: [w349 u32 0 ("Frame")] -> w4
    frame No Error {
      n93 = Unflatten From JSON(JSON string=w352, type and defaults=T21 {"Frame"=0, "Sensor Height"=0, "Sensor Width"=0, "ROI Height"=0, "ROI Width"=0, "ROI Enable?"=FALSE, "Bit per Pixel"=0} ("Camera IMAQ Key Info")) -> (value=w350:T21)  [unwired: 5 in, 1 out]
      n94 = Unbundle By Name(w350) -> ("Frame"=w349:u32)
    }
    frame Error {
    }
  }
  "Current Frame" <- w4
